vi "user process.vi"(8 "error in":errorcluster, 11 "Parameters to process":T2) -> (0 "error out":errorcluster, 3 "Results from processing":T1)   [LabVIEW 2014, in "LED runtime.lvclass"]
uses:
  LED runtime.lvclass
  parameter user data.ctl
  result user data.ctl
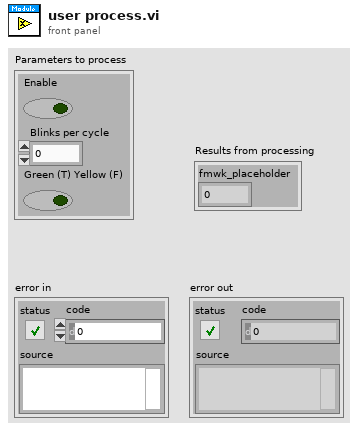
[diagram p1: front panel]
types:
  T1 = typedef "LED runtime.lvclass/result user data.ctl" = cluster{"fmwk_placeholder":i32}
  T2 = typedef "LED runtime.lvclass/parameter user data.ctl" = cluster{"Enable":bool, "Blinks per cycle":i32, "Green (T) Yellow (F)":bool}
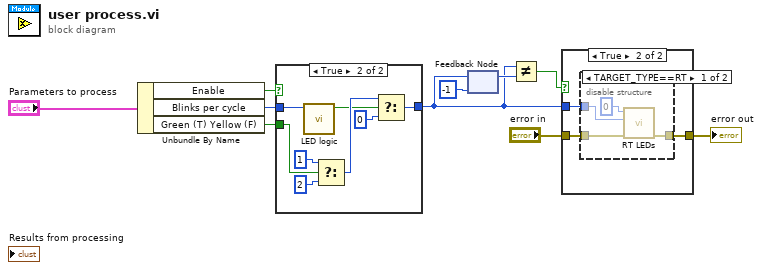
[diagram p0: block diagram]
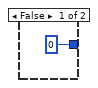
[diagram p4: hidden frame]
diagram:
  n1 = Unbundle By Name("Parameters to process") -> ("Enable"=w9:bool, "Blinks per cycle"=w7:i32, "Green (T) Yellow (F)"=w8:bool)
  n2 = case shown="True" w9 {
    tunnel: w8 -> [_ w19]
    tunnel: w7 -> [_ w13]
    tunnel: [0 ("f") w14] -> w2
    frame False {
    }
    frame True {
      n3 = call "LED logic.vi"("Blinks per cycle"=w13) -> ("Boolean"=w12:bool)  [unwired: 10 in]
      n4 = Select(t=1 ("State"), s=w19, f=2 ("State")) -> (s? t:f=w16:i32)
      n5 = Select(t=w16, s=w12, f=0) -> (s? t:f=w14:i32)
    }
  }
  n6 = feedback-in #1(w2) -> ()
  n7 = feedback #1(-1 ("f")) -> (w4:i32)
  n8 = Not Equal?(x=w2, y=w4) -> (x != y?=w3:bool)
  n9 = case shown="True" w3 {
    tunnel: [w20 w23] -> w6
    tunnel: "error in" -> [w20 w22]
    tunnel: w2 -> [_ w21]
    frame False {
    }
    frame True {
      n10 = disable-structure shown="TARGET_TYPE==RT" {
        disable-tunnel: w21 -> [w26 _]
        disable-tunnel: [w25 _] -> w23
        disable-tunnel: w22 -> [w24 _]
        frame condition #0 {
          n11 = call <vilib>:"RT LEDs.vi"("error in (no error)"=w24, "State"=w26, "LED Num"=0) -> ("error out"=w25:errorcluster)  [unwired: 3 in, 1 out]
        }
        frame condition #1 (active) {
        }
      }
    }
  }
  "error out" <- w6
